vi "Bnal BC table VI_MS.vi"(8 "error in":errorcluster, 10 "S New Info and MiN":T1={"Sample Sequence"="GATGATGATGATGATGAT", "Right Read MIN"=6, "Filter P"=0, "STD Type"=enum."Region", "Base Table"=[], "Selection"=enum."10kHz", "noise MAX"=3, "Sample name"="(GAT)x6"} {"Base Table"."Value 3" format="%.2g"}, 11 "Filename":path) -> (0 "error out":errorcluster, 3 "TDMSファイル out":refnum<k34>)   [LabVIEW 2018]
panel:
  out "BC Table":string[](array[string])
  out "BC Table Tag":string[](array[string])
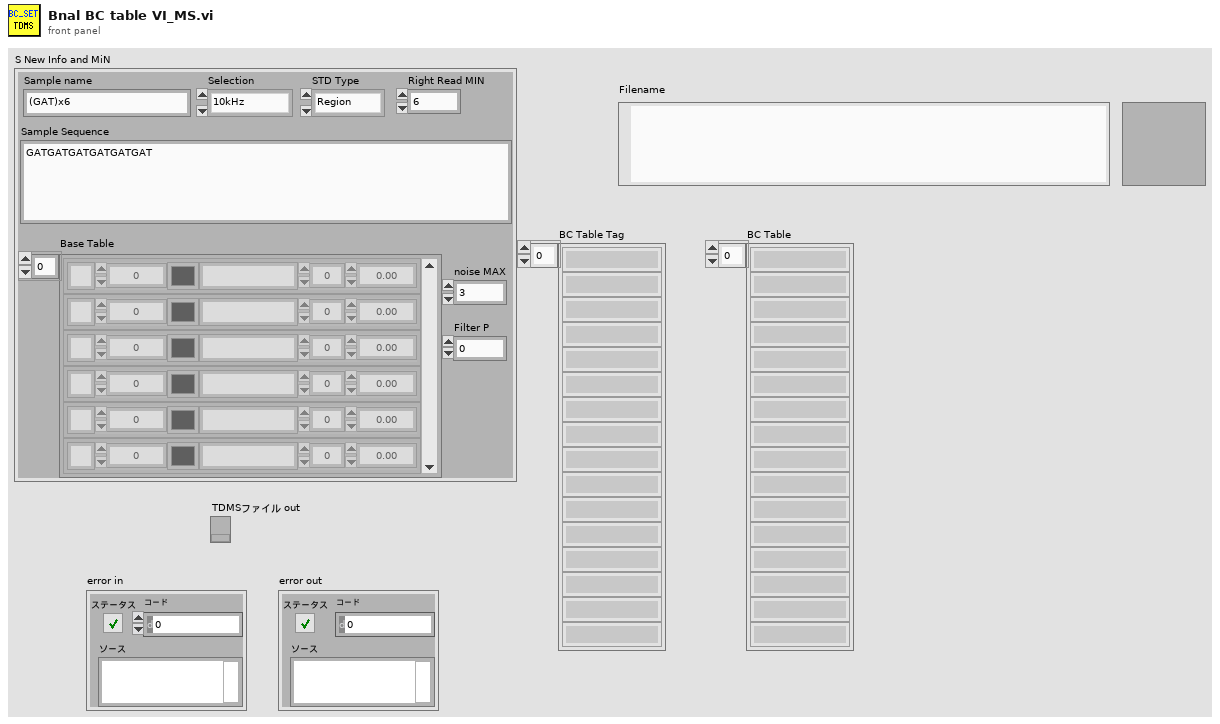
[diagram p1: front panel]
types:
  T1 = cluster{"Sample Sequence":string, "Right Read MIN":i32, "Filter P":i32, "STD Type":enum16{"Region", "Each", "Fixed"}, "Base Table":cluster{"Name":string, "Value":dbl, "Color":u32, "Name 2":string, "Value 2":dbl, "Value 3":dbl}[], "Selection":enum16{"10kHz", "100kHz"}, "noise MAX":i32, "Sample name":string}
  T2 = enum16{"open", "open or create", "create or replace", "create", "open (read-only)"}
  T3 = cluster{"Name":string, "Value":dbl, "Color":u32, "Name 2":string, "Value 2":dbl, "Value 3":dbl}[]
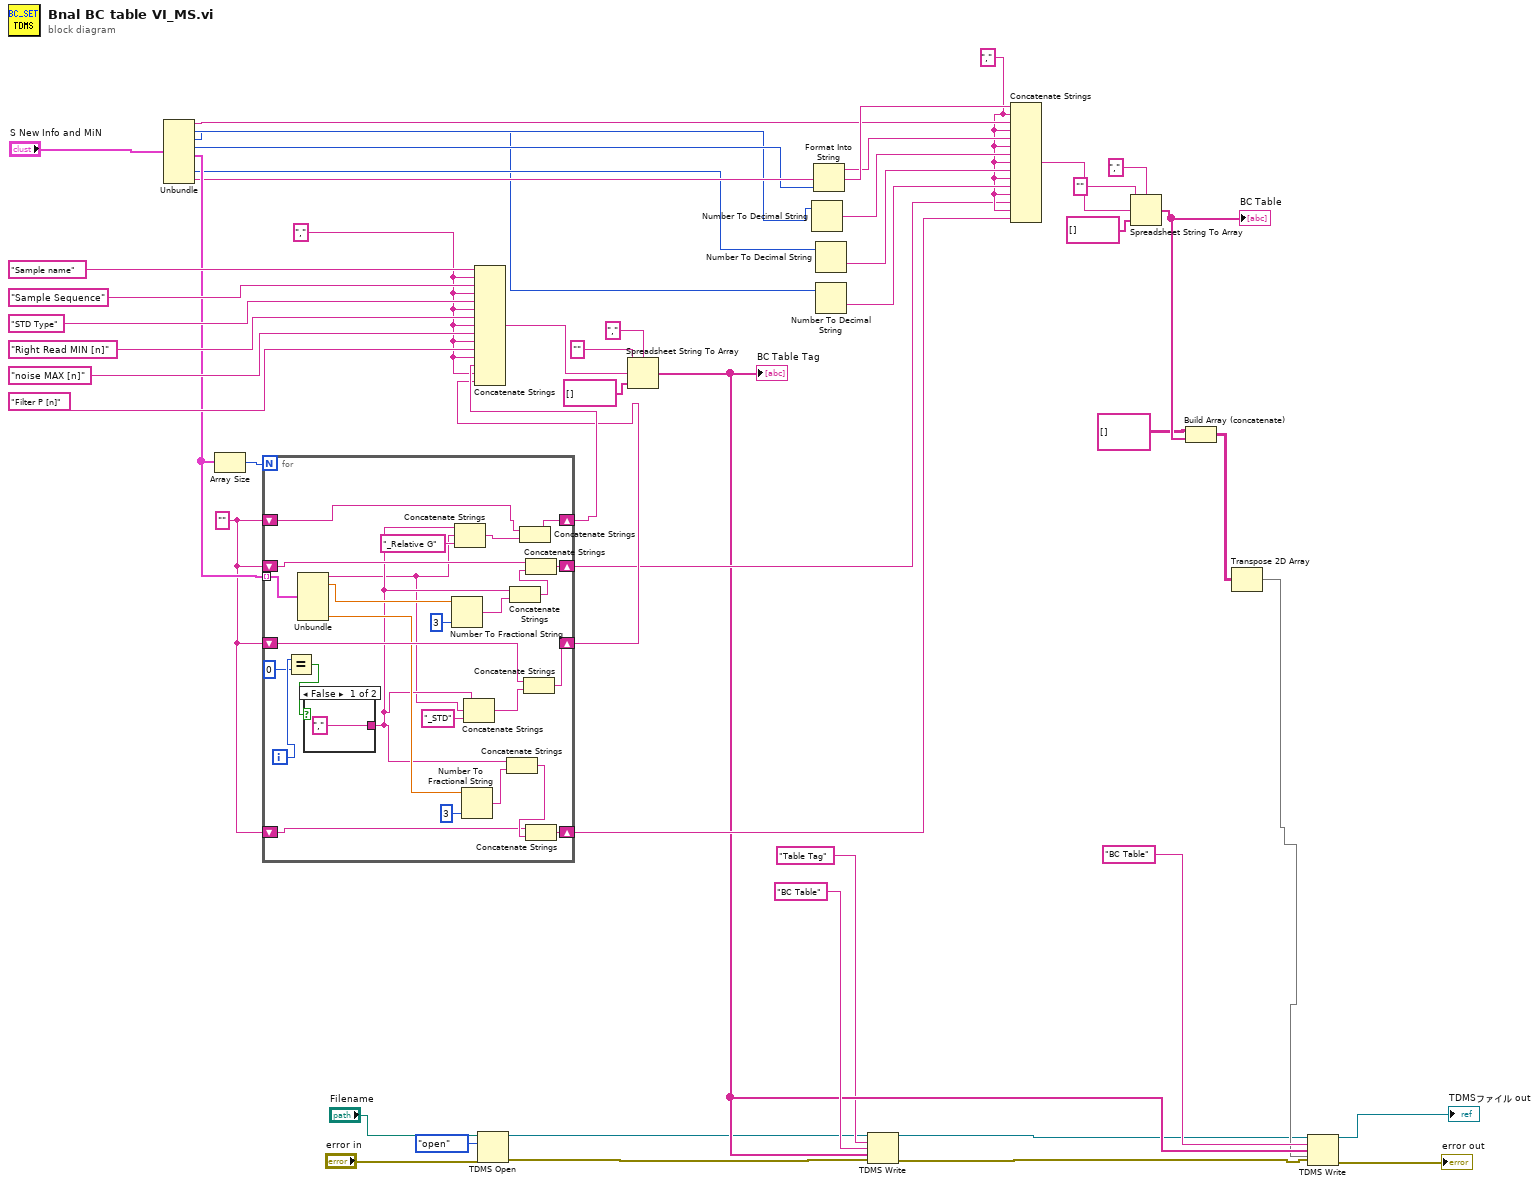
[diagram p0: block diagram]
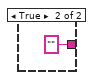
[diagram p2: hidden frame]
diagram:
  w21 = "," ("デリミタ（タブ）")
  w10 = ""
  w38 = "," ("デリミタ（タブ）")
  n1 = Unbundle("S New Info and MiN") -> ("Sample Sequence"=w30:string, "Right Read MIN"=w27:i32, "Filter P"=w23:i32, "STD Type"=w29:enum16{"Region", "Each", "Fixed"}, "Base Table"=w36:T3, "noise MAX"=w25:i32, "Sample name"=w31:string)  [unwired: 1 out]
  n2 = Array Size(array=w36) -> (size(s)=w40:i32)
  n3 = for {
    N: w40 -> [_]
    tunnel: w36 -> [w77] mode=indexing
    shift-right: [w71] -> w39
    shift-left: w10 -> [w70]
    shift-right: [w65] -> w37
    shift-left: w10 -> [w64]
    shift-right: [w61] -> w20
    shift-left: w10 -> [w60]
    shift-right: [w55] -> w19
    shift-left: w10 -> [w54]
    i -> [w69]
    n4 = Equal?(x=w69, y=0) -> (x = y?=w68:bool)
    n5 = Unbundle(w77) -> ("Name"=w52:string, "Value"=w76:dbl, "Value 3"=w58:dbl)  [unwired: 3 out]
    n6 = case shown="False" w68 {
      tunnel: ["," ("デリミタ（タブ）") "" ("デリミタ（タブ）")] -> w53
      frame False {
      }
      frame True {
      }
    }
    n7 = Number To Fractional String(number=w76, precision (6)=i16 3 ("精度（6）")) -> (F-format string=w63:string)  [unwired: 2 in]
    n8 = Concatenate Strings(w53, w52, "_Relative G" ("文字列")) -> (w72:string)
    n9 = Number To Fractional String(number=w58, precision (6)=i16 3 ("精度（6）")) -> (F-format string=w57:string)  [unwired: 2 in]
    n10 = Concatenate Strings(w53, w52, "_STD" ("文字列")) -> (w66:string)
    n11 = Concatenate Strings(w53, w57) -> (w56:string)
    n12 = Concatenate Strings(w53, w63) -> (w62:string)
    n13 = Concatenate Strings(w70, w72) -> (w71:string)
    n14 = Concatenate Strings(w64, w66) -> (w65:string)
    n15 = Concatenate Strings(w60, w62) -> (w61:string)
    n16 = Concatenate Strings(w54, w56) -> (w55:string)
  }
  n17 = Concatenate Strings("Sample name" ("文字列"), w38, "Sample Sequence" ("文字列"), w38, "STD Type" ("文字列"), w38, "Right Read MIN [n]" ("文字列"), w38, "noise MAX [n]" ("文字列"), w38, "Filter P [n]" ("文字列"), w38, w39, w38, w37) -> (w46:string)
  n18 = TDMS Open(8:"error in", 10:T2."open" ("操作（0:open）"), 11:"Filename") -> (0:w6:errorcluster, 3:w4:refnum<k34>)  [unwired: 4 in]
  n19 = Spreadsheet String To Array(delimiter (Tab)="," ("デリミタ（タブ）"), format string="" ("形式文字列"), spreadsheet string=w46, array type (2D Dbl)=string[] [] ("行ヘッダ文字列[]")) -> (array=w16:string[])
  "BC Table Tag" <- w16
  n20 = Number To Decimal String(number=w27) -> (decimal integer string=w26:string)  [unwired: 1 in]
  n21 = Format Into String(w29) -> (resulting string=w28:string)  [unwired: 3 in, 1 out]
  n22 = Number To Decimal String(number=w25) -> (decimal integer string=w24:string)  [unwired: 1 in]
  n23 = Number To Decimal String(number=w23) -> (decimal integer string=w22:string)  [unwired: 1 in]
  n24 = TDMS Write(0:w4, 5:"Table Tag" ("グループ名入力（名称未設定）"), 7:"BC Table" ("Group name"), 9:w16, 11:w6) -> (4:w1:refnum<k34>, 15:w2:errorcluster)  [unwired: 1 in, 2 out]
  n25 = Concatenate Strings(w31, w21, w30, w21, w28, w21, w26, w21, w24, w21, w22, w21, w20, w21, w19) -> (w32:string)
  n26 = Spreadsheet String To Array(delimiter (Tab)="," ("デリミタ（タブ）"), format string="" ("形式文字列"), spreadsheet string=w32, array type (2D Dbl)=string[] [] ("行ヘッダ文字列[]")) -> (array=w13:string[])
  "BC Table" <- w13
  n27 = Build Array (concatenate)(string[][] [] ("Table"), w13) -> (w12:string[][])
  n28 = Transpose 2D Array(2D array=w12) -> (transposed array=w14:string[][])
  n29 = TDMS Write(0:w1, 5:"BC Table" ("Group name"), 7:w16, 9:w14, 11:w2) -> (4:→"TDMSファイル out":refnum<k34>, 15:→"error out":errorcluster)  [unwired: 1 in, 2 out]
